vi "Max Scale Number--constant.vi"() -> (3 "Max Scale Number":i32)   [LabVIEW 2020, in "Data Viewer.lvlib"]
uses:
  Data Viewer.lvlib
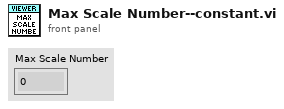
[diagram p1: front panel]
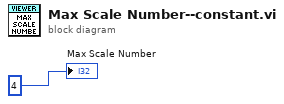
[diagram p0: block diagram]
diagram:
  "Max Scale Number" <- 4 ("y")
